vi "Read Numeric Input.vi"(8 "error in (no error)":errorcluster, 10 "Numeric Input in":T1, 11 "Modbus in":refnum<class "Modbus.lvclass">) -> (0 "error out":errorcluster, 2 "Numeric Value":dbl, 3 "Modbus out":refnum<class "Modbus.lvclass">)   [LabVIEW 2026, in "Modbus.lvlib" / "Modbus.lvclass"]
uses:
  Modbus.lvclass
  Types/Numeric Data.ctl
  Types/Modbus Table.ctl
  Types/Numeric Size.ctl
  Types/Numeric Data Type.ctl
  Types/Numeric Location.ctl
  Modbus.lvclass/Modbus.ctl
  <vilib>/ni/Modbus Library/API/Master/Modbus Master.lvclass
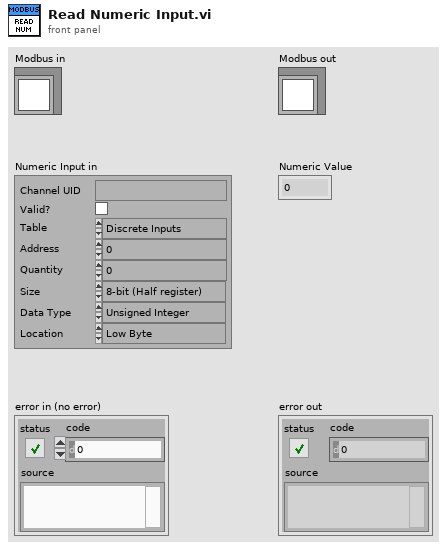
[diagram p1: front panel]
types:
  T1 = typedef "Modbus.lvlib/Modbus.lvclass/Numeric Data.ctl" = cluster{"Channel UID":string, "Valid?":bool, "Table":T2, "Address":i32, "Quantity":u16, "Size":T3, "Data Type":T4, "Location":T5}
  T2 = typedef "Modbus.lvlib/Modbus.lvclass/Modbus Table.ctl" = enum16{"Discrete Inputs", "Coils", "Input Registers", "Holding Registers"}
  T3 = typedef "Modbus.lvlib/Modbus.lvclass/Numeric Size.ctl" = enum16{"8-bit (Half register)", "16-bit (One register)", "32-bit (Two registers)", "64-bit (Four registers)"}
  T4 = typedef "Modbus.lvlib/Modbus.lvclass/Numeric Data Type.ctl" = enum16{"Unsigned Integer", "Signed Integer", "Floating Point"}
  T5 = typedef "Modbus.lvlib/Modbus.lvclass/Numeric Location.ctl" = enum16{"Low Byte", "High Byte"}
  T6 = typedef "Modbus.lvlib/Modbus.lvclass/Order.ctl" = enum16{"Big-Endian (AB CD)", "Word-Swap (CD AB)", "Byte-Swap (BA DC)", "Little-Endian (DC BA)"}
  T7 = typedef "Utility.lvlib/Signed Representation.ctl" = enum16{"Two's Complement", "Offset Binary", "Sign-Magnitude", "Ones' Complement"}
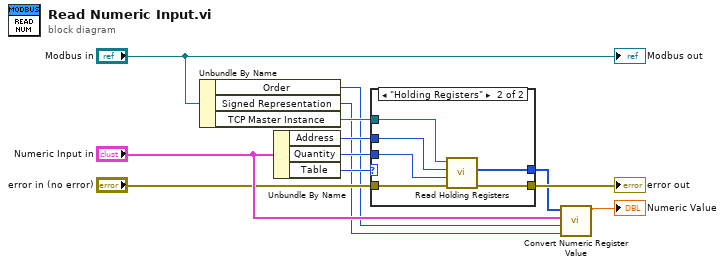
[diagram p0: block diagram]
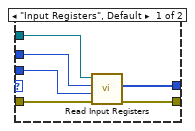
[diagram p2: hidden frame]
diagram:
  n1 = Unbundle By Name("Modbus in") -> ("Order"=w2:T6, "Signed Representation"=w1:T7, "TCP Master Instance"=w6:refnum<class "Modbus Master.lvclass">)
  n2 = Unbundle By Name("Numeric Input in") -> ("Address"=w5:i32, "Quantity"=w4:u16, "Table"=w3:T2)
  n3 = case shown="\"Holding Registers\"" w3 {
    tunnel: w6 -> [w18 w24]
    tunnel: [w17 w23] -> w10
    tunnel: w5 -> [w16 w22]
    tunnel: [w15 w21] -> w7
    tunnel: w4 -> [w14 w20]
    tunnel: "error in (no error)" -> [w13 w19]
    frame "Input Registers", Default {
      n4 = call-dynamic "Read Input Registers.vi"("error in"=w13, "number of inputs"=w14, "starting address"=w16, "Modbus master in"=w18) -> ("error out"=w17:errorcluster, "register values"=w15:u16[])  [unwired: 5 in, 1 out]
    }
    frame "Holding Registers" {
      n5 = call-dynamic "Read Holding Registers.vi"("error in"=w19, "number of inputs"=w20, "starting address"=w22, "Modbus master in"=w24) -> ("error out"=w23:errorcluster, "register values"=w21:u16[])  [unwired: 5 in, 1 out]
    }
  }
  "error out" <- w10
  n6 = call "Convert Numeric Register Value.vi"("Signed representation"=w1, "Order"=w2, "Numeric Input"="Numeric Input in", "Register Values"=w7) -> ("Number out"=→"Numeric Value":dbl)  [unwired: 7 in]
  "Modbus out" <- "Modbus in"
